vi "PhotonTrackedTarget_Equals.vi"(9 "Other TrackedTarget":T1={"Yaw"=0.0, "Pitch"=0.0, "Area"=0.0, "Skew"=0.0, "TargetCorners"=[], "CameraToTarget"={"TRANSLATION"={"X"=0.0, "Y"=0.0}, "ROTATION"={"VALUE"=0.0, "COS"=1.0, "SIN"=0.0}}} {"CameraToTarget"."ROTATION"."SIN" format="%13.4f"; "CameraToTarget"."ROTATION"."COS" format="%13.4f"; "CameraToTarget"."ROTATION"."VALUE" format="%13.4f"; "CameraToTarget"."TRANSLATION"."Y" format="%14.3f"; "CameraToTarget"."TRANSLATION"."X" format="%14.3f"}, 11 "TrackedTarget":T1={"Yaw"=0.0, "Pitch"=0.0, "Area"=0.0, "Skew"=0.0, "TargetCorners"=[], "CameraToTarget"={"TRANSLATION"={"X"=0.0, "Y"=0.0}, "ROTATION"={"VALUE"=0.0, "COS"=1.0, "SIN"=0.0}}} {"CameraToTarget"."ROTATION"."SIN" format="%13.4f"; "CameraToTarget"."ROTATION"."COS" format="%13.4f"; "CameraToTarget"."ROTATION"."VALUE" format="%13.4f"; "CameraToTarget"."TRANSLATION"."Y" format="%14.3f"; "CameraToTarget"."TRANSLATION"."X" format="%14.3f"}) -> (3 "Equals":bool)   [LabVIEW 2019, in "PhotonVisionLib.lvlib"]
doc: "Determines if two tracked targets are equal\n\nInputs:\n - TrackedTarget -- TrackedTarget cluster.\n - OtherTrackedTarget -- Second TrackedTarget cluster.\n\nOutputs:\n - Area -- Boolean, equals TRUE if both TrackedTargets are the same."
uses:
  TypeDef/PhotonTrackedTargetType.ctl
  TypeDef/TargetCornerType.ctl
  <vilib>/Rock Robotics/WPI/ThirdParty/JAS_Junk/TrajLib/TRANSFORM2D.ctl
  <vilib>/Rock Robotics/WPI/ThirdParty/JAS_Junk/TrajLib/TRANSLATION2D.ctl
  <vilib>/Rock Robotics/WPI/ThirdParty/JAS_Junk/TrajLib/ROTATION2D.ctl
  PhotonVisionLib.lvlib
  <vilib>/Rock Robotics/WPI/ThirdParty/JAS_Junk/TrajLib/Trajectory_Library.lvlib
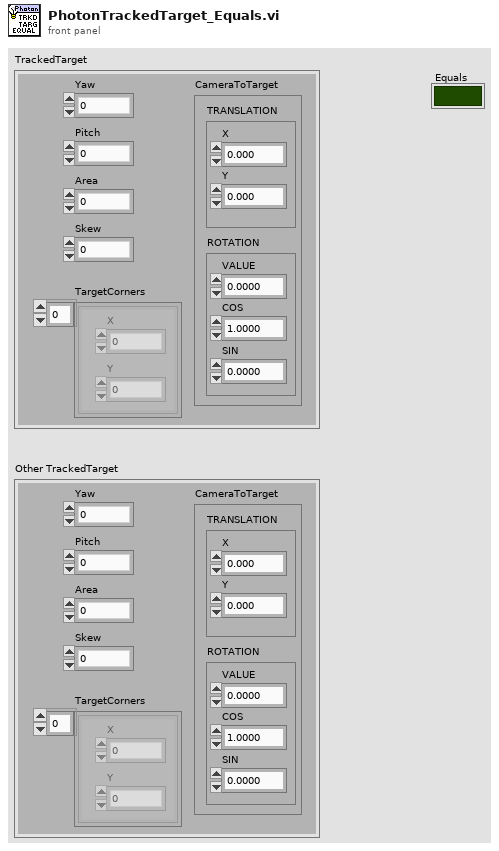
[diagram p1: front panel]
types:
  T1 = typedef "PhotonVisionLib.lvlib/PhotonTrackedTargetType.ctl" = cluster{"Yaw":dbl, "Pitch":dbl, "Area":dbl, "Skew":dbl, "TargetCorners":T2[], "CameraToTarget":T3}
  T2 = typedef "PhotonVisionLib.lvlib/TargetCornerType.ctl" = cluster{"X":dbl, "Y":dbl}
  T3 = typedef "Trajectory_Library.lvlib/TRANSFORM2D.ctl" = cluster{"TRANSLATION":T4, "ROTATION":T5}
  T4 = typedef "Trajectory_Library.lvlib/TRANSLATION2D.ctl" = cluster{"X":dbl, "Y":dbl}
  T5 = typedef "Trajectory_Library.lvlib/ROTATION2D.ctl" = cluster{"VALUE":dbl, "COS":dbl, "SIN":dbl}
  T6 = cluster{"Yaw":bool, "Pitch":bool, "Area":bool, "Skew":bool, "TargetCorners":cluster{"X":bool, "Y":bool}[], "CameraToTarget":cluster{"TRANSLATION":cluster{"X":bool, "Y":bool}, "ROTATION":cluster{"VALUE":bool, "COS":bool, "SIN":bool}}}
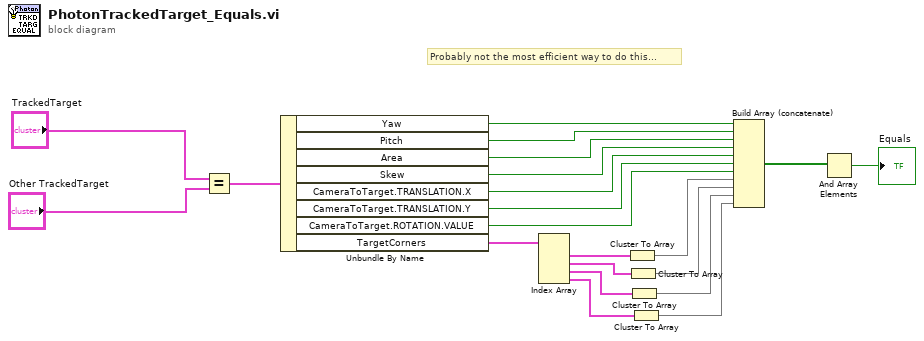
[diagram p0: block diagram]
diagram:
  # "Probably not the most efficient way to do this..."
  n1 = Equal?(x="TrackedTarget", y="Other TrackedTarget") -> (x = y?=w19:T6)
  n2 = Unbundle By Name(w19) -> ("Yaw"=w13:bool, "Pitch"=w12:bool, "Area"=w11:bool, "Skew"=w10:bool, "CameraToTarget.TRANSLATION.X"=w9:bool, "CameraToTarget.TRANSLATION.Y"=w8:bool, "CameraToTarget.ROTATION.VALUE"=w7:bool, "TargetCorners"=w18:cluster{"X":bool, "Y":bool}[])
  n3 = Index Array(array=w18) -> (element #1=w17:cluster{"X":bool, "Y":bool}, element #2=w16:cluster{"X":bool, "Y":bool}, element #3=w15:cluster{"X":bool, "Y":bool}, element #4=w14:cluster{"X":bool, "Y":bool})  [unwired: 4 in]
  n4 = Cluster To Array(cluster=w17) -> (array=w6:bool[])
  n5 = Cluster To Array(cluster=w16) -> (array=w5:bool[])
  n6 = Cluster To Array(cluster=w15) -> (array=w4:bool[])
  n7 = Cluster To Array(cluster=w14) -> (array=w3:bool[])
  n8 = Build Array (concatenate)(w13, w12, w11, w10, w9, w8, w7, w6, w5, w4, w3) -> (w2:bool[])
  n9 = And Array Elements(Boolean array=w2) -> (logical AND=→"Equals":bool)
